vi "measure BT Tescom xDB.vi"(8 "error in (no error)":errorcluster, 11 "SA Measurement in":refnum<class "SA Measurement.lvclass">) -> (0 "error out":errorcluster, 3 "SA Measurement out":refnum<class "SA Measurement.lvclass">)   [LabVIEW 2023, in "Spectrum Analyzer.lvlib" / "SA Measurement.lvclass"]
uses:
  SA Measurement.lvclass
  SA Measurement.lvclass/SA Measurement.ctl
  TYPE DEFINITION/Keysight 9020A/TYPE Measurement Preset.ctl
  Spectrum Analyzer.lvlib
  TYPE DEFINITION/TYPE RBW and VBW Select.ctl
  TYPE DEFINITION/TYPE Marker Peak Search Type.ctl
  Interface_Spectrum/Interface_Spectrum.lvclass
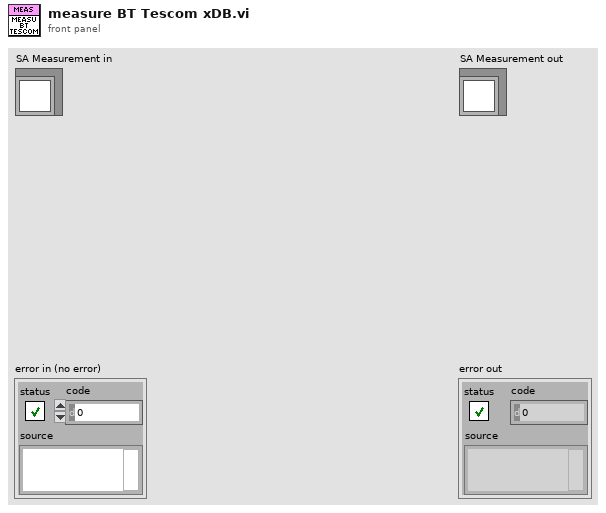
[diagram p1: front panel]
types:
  T1 = typedef "Spectrum Analyzer.lvlib/TYPE Marker Peak Search Type.ctl" = enum16{"Max", "Next Peak"}
  T2 = typedef "Spectrum Analyzer.lvlib/TYPE RBW and VBW Select.ctl" = enum16{"Res BW", "Video BW"}
  T3 = typedef "Spectrum Analyzer.lvlib/TYPE Measurement Preset.ctl" = enum16{"Sweep SA Mode", "Channel Power", "Occupied BW", "ACP", "Spurious Emission", "Spurious Emission Mask", "Burst Power (Transmit Power)"}
  T4 = typedef "Spectrum Analyzer.lvlib/TYPE Y-axis Unit.ctl" = enum16{"dBm", "dBmV", "dBuV", "dBpW", "Volt", "Ampere", "Watt"}
  T5 = typedef "Spectrum Analyzer.lvlib/TYPE Reference Level and Atten Param.ctl" = cluster{"Reference Level":dbl, "Atten":i32, "Atten Auto?":bool, "Reference Level Offset":dbl}
  T6 = typedef "Spectrum Analyzer.lvlib/TYPE Display Trace Mode Select.ctl" = enum16{"Clear Write", "Max Hold", "Min Hold", "Average", "View"}
  T7 = typedef "Spectrum Analyzer.lvlib/TYPE Detect Mode Select.ctl" = enum16{"Det Auto (Normal)", "Auto Peak", "Positive Peak", "Negative Peak", "Sample", "RMS", "Average", "Quasipeak", "CISPR Average", "RMS Average"}
  T8 = cluster{"Trace Mode":T6, "Detector Type":T7, "Detect Auto?":bool}[]
  T9 = typedef "Spectrum Analyzer.lvlib/TYPE OBW Measurement.ctl" = cluster{"Occupied BW (Hz)":dbl, "Total Power or OBW Power - dBm":dbl, "Transmit Frequency Error (Hz)":dbl, "x DB Bandwidth (Hz)":dbl, "Lower OBW Frequency (Hz)":dbl, "Upper OBW Frequency (Hz)":dbl}
  T10 = typedef "Spectrum Analyzer.lvlib/TYPE Marker Value.ctl" = cluster{"X-axis":dbl, "Y-axis":dbl}
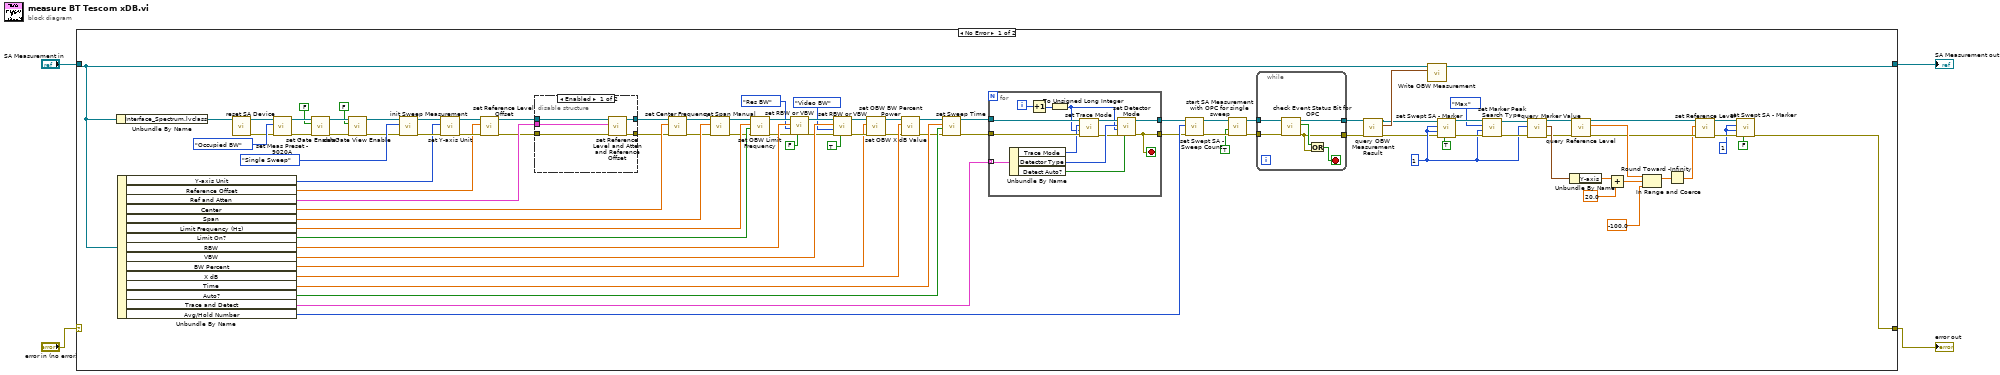
[diagram p0: block diagram]
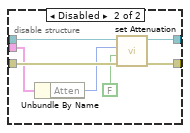
[diagram p2: hidden frame]
diagram:
  n1 = case shown="No Error" "error in (no error)" {
    selector: "error in (no error)" -> [_ w131]
    tunnel: [w23 w131] -> w1
    tunnel: [w49 w130] -> w2
    tunnel: "SA Measurement in" -> [w51 w130]
    frame No Error {
      w24 = 1 ("Index")
      w42 = 1 ("Index")
      n2 = Unbundle By Name(w51) -> ("Interface_Spectrum.lvclass"=w84:refnum<class "Interface_Spectrum.lvclass">)
      n3 = Unbundle By Name(w51) -> ("Y-axis Unit"=w92:T4, "Reference Offset"=w12:dbl, "Ref and Atten"=w96:T5, "Center"=w95:dbl, "Span"=w77:dbl, "Limit Frequency (Hz)"=w81:dbl, "Limit On?"=w80:bool, "RBW"=w72:dbl, "VBW"=w66:dbl, "BW Percent"=w7:dbl, "X dB"=w79:dbl, "Time"=w62:dbl, "Auto?"=w61:bool, "Trace and Detect"=w91:T8, "Avg/Hold Number"=w90:u32)
      n4 = call-dynamic "reset SA Device.vi"("Interface_Spectrum in"=w84) -> ("error out"=w82:errorcluster, "Interface_Spectrum out"=w83:refnum<class "Interface_Spectrum.lvclass">)  [unwired: 9 in]
      n5 = call-dynamic "set Meas Preset - 9020A.vi"("error in (no error)"=w82, "Measurement Preset"=TYPE_Measurement_Preset."Occupied BW", "Interface_Spectrum in"=w83) -> ("error out"=w21:errorcluster, "Interface_Spectrum out"=w22:refnum<class "Interface_Spectrum.lvclass">)  [unwired: 7 in]
      n6 = call-dynamic "set Gate Enable.vi"("error in (no error)"=w21, "Gate Enable"=FALSE, "Interface_Spectrum in"=w22) -> ("error out"=w18:errorcluster, "Interface_Spectrum out"=w19:refnum<class "Interface_Spectrum.lvclass">)  [unwired: 7 in]
      n7 = call-dynamic "set Gate View Enable.vi"("error in (no error)"=w18, "Gate View Enable"=FALSE, "Interface_Spectrum in"=w19) -> ("error out"=w15:errorcluster, "Interface_Spectrum out"=w16:refnum<class "Interface_Spectrum.lvclass">)  [unwired: 7 in]
      n8 = call-dynamic "init Sweep Measurement.vi"("error in (no error)"=w15, "Sweep Measurement Mode"=enum16{"Single Sweep", "Continuous Sweep"}."Single Sweep", "Interface_Spectrum in"=w16) -> ("error out"=w93:errorcluster, "Interface_Spectrum out"=w94:refnum<class "Interface_Spectrum.lvclass">)  [unwired: 7 in]
      n9 = call-dynamic "set Y-axis Unit.vi"("error in (no error)"=w93, "Y-axis Unit"=w92, "Interface_Spectrum in"=w94) -> ("error out"=w13:errorcluster, "Interface_Spectrum out"=w14:refnum<class "Interface_Spectrum.lvclass">)  [unwired: 7 in]
      n10 = call-dynamic "set Reference Level Offset.vi"("error in (no error)"=w13, "Reference Level Offset"=w12, "Interface_Spectrum in"=w14) -> ("error out"=w10:errorcluster, "Interface_Spectrum out"=w11:refnum<class "Interface_Spectrum.lvclass">)  [unwired: 7 in]
      n11 = disable-structure shown="Enabled" {
        disable-tunnel: w96 -> [w103 w106]
        disable-tunnel: w11 -> [w102 w110]
        disable-tunnel: w10 -> [w101 w109]
        disable-tunnel: [w100 w108] -> w57
        disable-tunnel: [w99 w107] -> w56
        frame Enabled {
          n12 = call-dynamic "set Reference Level and Atten and Reference Offset.vi"("error in (no error)"=w101, "Reference Level, Atten, Reference Offset"=w103, "Interface_Spectrum in"=w102) -> ("error out"=w99:errorcluster, "Interface_Spectrum out"=w100:refnum<class "Interface_Spectrum.lvclass">)  [unwired: 7 in]
        }
        frame Disabled {
          n13 = Unbundle By Name(w106) -> ("Atten"=w105:i32)
          n14 = call-dynamic "set Attenuation.vi"("error in (no error)"=w109, "Auto?"=FALSE, "Attenuation"=w105, "Interface_Spectrum in"=w110) -> ("error out"=w107:errorcluster, "Interface_Spectrum out"=w108:refnum<class "Interface_Spectrum.lvclass">)  [unwired: 6 in]
        }
      }
      n15 = call-dynamic "set Center Frequency.vi"("error in (no error)"=w56, "Center Frequency (Hz)"=w95, "Interface_Spectrum in"=w57) -> ("error out"=w76:errorcluster, "Interface_Spectrum out"=w78:refnum<class "Interface_Spectrum.lvclass">)  [unwired: 7 in]
      n16 = call-dynamic "set Span Manual.vi"("error in (no error)"=w76, "Span (Hz)"=w77, "Interface_Spectrum in"=w78) -> ("error out"=w74:errorcluster, "Interface_Spectrum out"=w75:refnum<class "Interface_Spectrum.lvclass">)  [unwired: 7 in]
      n17 = call-dynamic "set OBW Limit Frequency.vi"("error in (no error)"=w74, "Limit On?"=w80, "Limit Frequency (Hz)"=w81, "Interface_Spectrum in"=w75) -> ("error out"=w70:errorcluster, "Interface_Spectrum out"=w73:refnum<class "Interface_Spectrum.lvclass">)  [unwired: 6 in]
      n18 = call-dynamic "set RBW or VBW.vi"("BW Auto?"=FALSE, "error in (no error)"=w70, "BW Type"=TYPE_RBW_and_VBW_Select."Res BW", "BW Value (Hz)"=w72, "Interface_Spectrum in"=w73) -> ("error out"=w64:errorcluster, "Interface_Spectrum out"=w67:refnum<class "Interface_Spectrum.lvclass">)  [unwired: 5 in]
      n19 = call-dynamic "set RBW or VBW.vi"("BW Auto?"=TRUE, "error in (no error)"=w64, "BW Type"=TYPE_RBW_and_VBW_Select."Video BW", "BW Value (Hz)"=w66, "Interface_Spectrum in"=w67) -> ("error out"=w8:errorcluster, "Interface_Spectrum out"=w9:refnum<class "Interface_Spectrum.lvclass">)  [unwired: 5 in]
      n20 = call-dynamic "set OBW BW Percent Power.vi"("error in (no error)"=w8, "OBW BW % Pwr"=w7, "Interface_Spectrum in"=w9) -> ("error out"=w5:errorcluster, "Interface_Spectrum out"=w6:refnum<class "Interface_Spectrum.lvclass">)  [unwired: 7 in]
      n21 = call-dynamic "set OBW X dB Value.vi"("error in (no error)"=w5, "OBW X dB (minus Value)"=w79, "Interface_Spectrum in"=w6) -> ("error out"=w60:errorcluster, "Interface_Spectrum out"=w63:refnum<class "Interface_Spectrum.lvclass">)  [unwired: 7 in]
      n22 = call-dynamic "set Sweep Time.vi"("error in (no error)"=w60, "Sweep Time Auto?"=w61, "Sweep Time(sec)"=w62, "Interface_Spectrum in"=w63) -> ("error out"=w58:errorcluster, "Interface_Spectrum out"=w59:refnum<class "Interface_Spectrum.lvclass">)  [unwired: 6 in]
      n23 = for {
        tunnel: w59 -> [w128]
        tunnel: w58 -> [w127]
        tunnel: w91 -> [w129] mode=indexing
        tunnel: [w117] -> w54
        tunnel: [w118] -> w55
        i -> [w126]
        stop <- w117 stop-if-true
        n24 = Unbundle By Name(w129) -> ("Trace Mode"=w124:T6, "Detector Type"=w122:T7, "Detect Auto?"=w119:bool)
        n25 = Increment(x=w126) -> (x+1=w125:i32)
        n26 = To Unsigned Long Integer(number=w125) -> (unsigned 32bit integer=w120:u32)
        n27 = call-dynamic "set Trace Mode.vi"("error in (no error)"=w127, "Trace Index"=w120, "Trace Mode"=w124, "Interface_Spectrum in"=w128) -> ("error out"=w121:errorcluster, "Interface_Spectrum out"=w123:refnum<class "Interface_Spectrum.lvclass">)  [unwired: 6 in]
        n28 = call-dynamic "set Detector Mode.vi"("Detect Auto?"=w119, "error in (no error)"=w121, "Trace Index"=w120, "Detector Type"=w122, "Interface_Spectrum in"=w123) -> ("error out"=w117:errorcluster, "Interface_Spectrum out"=w118:refnum<class "Interface_Spectrum.lvclass">)  [unwired: 5 in]
      }
      n29 = call-dynamic "set Swept SA - Sweep Count.vi"("error in (no error)"=w54, "Sweep Count"=w90, "Interface_Spectrum in"=w55) -> ("error out"=w88:errorcluster, "Interface_Spectrum out"=w89:refnum<class "Interface_Spectrum.lvclass">)  [unwired: 7 in]
      n30 = call-dynamic "start SA Measurement with OPC for single sweep.vi"("error in (no error)"=w88, "with OPC?"=TRUE, "Interface_Spectrum in"=w89) -> ("error out"=w85:errorcluster, "Interface_Spectrum out"=w86:refnum<class "Interface_Spectrum.lvclass">)  [unwired: 7 in]
      n31 = while {
        tunnel: w86 -> [w116]
        tunnel: w85 -> [w115]
        tunnel: [w112] -> w52
        tunnel: [w111] -> w53
        stop <- w113 stop-if-true
        n32 = call-dynamic "check Event Status Bit for OPC.vi"("error in (no error)"=w115, "Interface_Spectrum in"=w116) -> ("error out"=w112:errorcluster, "OPC Bit Changed?"=w114:bool, "Interface_Spectrum out"=w111:refnum<class "Interface_Spectrum.lvclass">)  [unwired: 7 in]
        n33 = Or(x=w114, y=w112) -> (x .or. y?=w113:bool)
      }
      n34 = call-dynamic "query OBW Measurement Result.vi"("error in (no error)"=w52, "Interface_Spectrum in"=w53) -> ("error out"=w28:errorcluster, "OBW Measurement"=w50:T9, "Interface_Spectrum out"=w29:refnum<class "Interface_Spectrum.lvclass">)  [unwired: 7 in]
      n35 = call "Write OBW Measurement.vi"("OBW Measurement"=w50, "SA Measurement in"=w51) -> ("SA Measurement out"=w49:refnum<class "SA Measurement.lvclass">)  [unwired: 8 in, 1 out]
      n36 = call-dynamic "set Swept SA - Marker.vi"("On?"=TRUE, "error in (no error)"=w28, "trace"=w42, "Index"=w42, "Interface_Spectrum in"=w29) -> ("error out"=w46:errorcluster, "Interface_Spectrum out"=w47:refnum<class "Interface_Spectrum.lvclass">)  [unwired: 5 in]
      n37 = call-dynamic "set Marker Peak Search Type.vi"("error in (no error)"=w46, "Marker Index"=w42, "Peak Search Type"=TYPE_Marker_Peak_Search_Type."Max", "Interface_Spectrum in"=w47) -> ("error out"=w43:errorcluster, "Interface_Spectrum out"=w44:refnum<class "Interface_Spectrum.lvclass">)  [unwired: 6 in]
      n38 = call-dynamic "query Marker Value.vi"("error in (no error)"=w43, "Marker Index"=w42, "Interface_Spectrum in"=w44) -> ("error out"=w37:errorcluster, "Marker Value"=w39:T10, "Interface_Spectrum out"=w38:refnum<class "Interface_Spectrum.lvclass">)  [unwired: 6 in]
      n39 = Unbundle By Name(w39) -> ("Y-axis"=w41:dbl)
      n40 = call-dynamic "query Reference Level.vi"("error in (no error)"=w37, "Interface_Spectrum in"=w38) -> ("error out"=w32:errorcluster, "Ref Level"=w35:dbl, "Interface_Spectrum out"=w36:refnum<class "Interface_Spectrum.lvclass">)  [unwired: 7 in]
      n41 = Add(x=w41, y=20.0) -> (x+y=w34:dbl)
      n42 = In Range and Coerce(upper limit=w35, x=w34, lower limit=-100.0) -> (coerced(x)=w31:dbl)  [unwired: 1 out]
      n43 = Round Toward -Infinity(1:w31) -> (0:w30:dbl)
      n44 = call-dynamic "set Reference Level.vi"("error in (no error)"=w32, "Reference Level"=w30, "Interface_Spectrum in"=w36) -> ("error out"=w26:errorcluster, "Interface_Spectrum out"=w27:refnum<class "Interface_Spectrum.lvclass">)  [unwired: 7 in]
      n45 = call-dynamic "set Swept SA - Marker.vi"("On?"=FALSE, "error in (no error)"=w26, "trace"=w24, "Index"=w24, "Interface_Spectrum in"=w27) -> ("error out"=w23:errorcluster)  [unwired: 5 in, 1 out]
    }
    frame Error {
    }
  }
  "error out" <- w1
  "SA Measurement out" <- w2
